vi "CSE routine - Load FuncVIs.vi"(5 "test arg num":bool, 6 "error in":errorcluster, 7 "FuncVIs info":string[](array[string]), 9 "CSE RefNum":T1) -> (0 "error out":errorcluster, 2 "loaded functions":string[](array[string]))   [LabVIEW 2021]
doc: "::: CalcExpress Toolkit :::\nCopyright (c) 2000-2026 Konstantin Shifershteyn. All rights reserved."
uses:
  CSE Instance RefNum.ctl
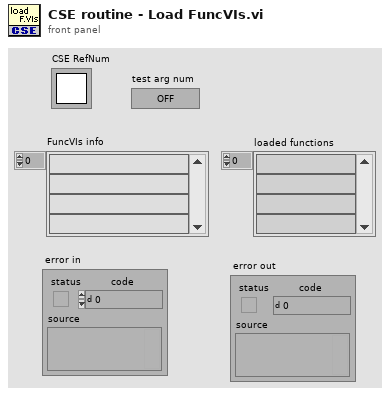
[diagram p1: front panel]
types:
  T1 = typedef "CSE Instance RefNum.ctl" = refnum<k1>
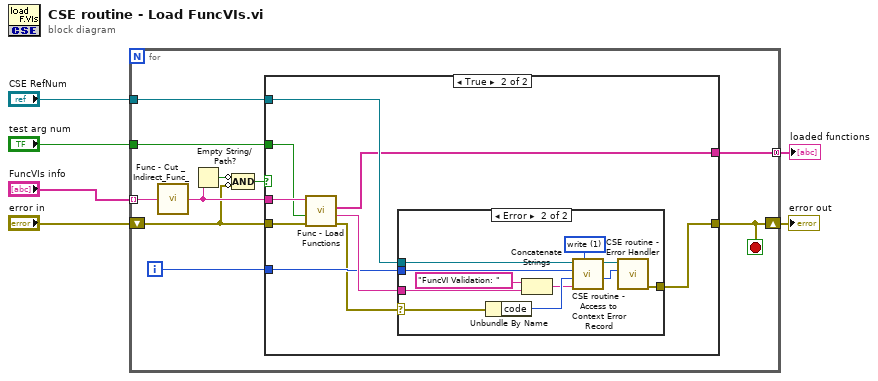
[diagram p0: block diagram]
diagram:
  n1 = for {
    tunnel: "FuncVIs info" -> [w14] mode=indexing
    shift-left: "error in" -> [w9]
    shift-right: [w8] -> w4
    tunnel: "test arg num" -> [w11]
    tunnel: "CSE RefNum" -> [w10]
    tunnel: [w7] -> w1 mode=concatenating
    i -> [w12]
    stop <- w8 stop-if-true
    n2 = call "Func - Cut _Indirect_Func_.vi"("FuncVI List"=w14) -> ("FuncVI List out"=w13:string)  [unwired: 4 in]
    n3 = Empty String/Path?(string/path=w13) -> (empty?=w16:bool)
    n4 = Compound Arithmetic op=AND(invert w16, invert w9) -> (w15:bool)
    n5 = case shown="True" w15 {
      tunnel: w9 -> [w17 w26]
      tunnel: [w17 w21] -> w8
      tunnel: w13 -> [_ w25]
      tunnel: w12 -> [_ w23]
      tunnel: w11 -> [_ w20]
      tunnel: w10 -> [_ w19]
      tunnel: [_ w18] -> w7
      frame False {
      }
      frame True {
        n6 = call "Func - Load Functions.vi"("error in"=w26, "test arg num (F)"=w20, "List of func names"=w25) -> ("error out"=w22:errorcluster, "error message"=w24:string, "loaded functions"=w18:string[])  [unwired: 4 in]
        n7 = case shown="Error" w22 {
          selector: w22 -> [w27 w37]
          tunnel: w24 -> [_ w36]
          tunnel: w23 -> [_ w34]
          tunnel: [w27 w31] -> w21
          tunnel: w19 -> [_ w28]
          frame No Error {
          }
          frame Error {
            w35 = 1 items=["read", "write", "reset"] ("cmd (0: read)")
            n8 = Unbundle By Name(w37) -> ("code"=w38:i32)
            n9 = Concatenate Strings("FuncVI Validation: " ("string"), w36) -> (w30:string)
            n10 = call "CSE routine - Access to Context Error Record.vi"("cmd (0: read)"=w35, "error message in"=w30, "error code in"=w38, "Stm Index in"=w34, "CSE RefNum"=w28) -> ("error code out"=w33:i32, "dup CSE RefNum"=w32:T1)  [unwired: 2 in, 3 out]
            n11 = call "CSE routine - Error Handler.vi"("exec status"=w33, "CSE RefNum"=w32) -> ("error out"=w31:errorcluster)  [unwired: 5 in, 2 out]
          }
        }
      }
    }
  }
  "error out" <- w4
  "loaded functions" <- w1
